vi "W08_T03_Judge.vi"() -> ()   [LabVIEW 2018]
doc: "Use this template to build a VI to use as a subVI."
panel:
  out "error out":errorcluster
  out "result":string
  out "value used":dbl
  in  "error in (no error)":errorcluster
  in  "true V (sim)":dbl
  in  "DMM loose (sim)":bool
  # "Read DMM.vi here is a fake (W08_sub). DMM loose (sim) and true V (sim) stand in for the real meter."
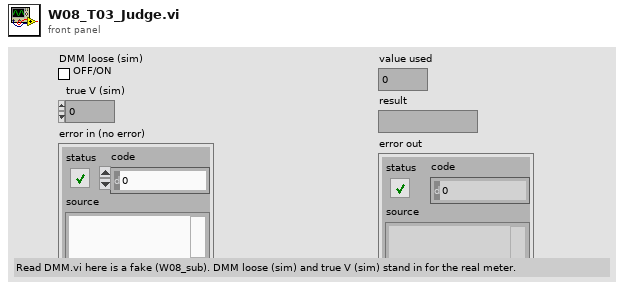
[diagram p1: front panel]
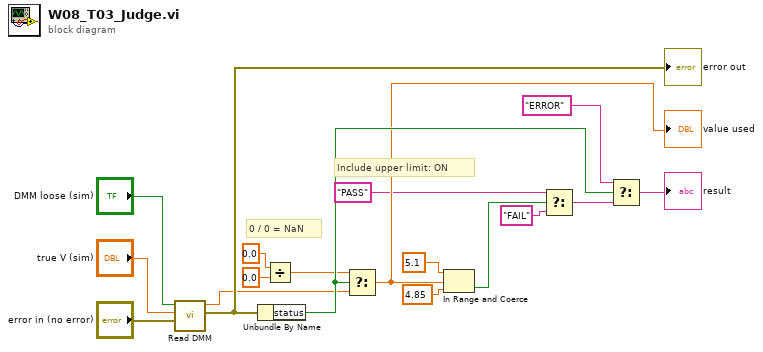
[diagram p0: block diagram]
diagram:
  # "Include upper limit: ON"
  # "0 / 0 = NaN"
  n1 = call "Read DMM.vi"("error in (no error)"="error in (no error)", "true V (sim)"="true V (sim)", "DMM loose (sim)"="DMM loose (sim)") -> ("error out"=w15:errorcluster, "reading"=w13:dbl)  [unwired: 7 in]
  "error out" <- w15
  n2 = Unbundle By Name(w15) -> ("status"=w14:bool)
  n3 = Divide(x=0.0, y=0.0) -> (x/y=w10:dbl)
  n4 = Select(t=w10, s=w14, f=w13) -> (s? t:f=w9:dbl)
  "value used" <- w9
  n5 = In Range and Coerce(upper limit=5.1, x=w9, lower limit=4.85) -> (In Range?=w6:bool)  [unwired: 1 out]
  n6 = Select(t="PASS", s=w6, f="FAIL") -> (s? t:f=w2:string)
  n7 = Select(t="ERROR", s=w14, f=w2) -> (s? t:f=→"result":string)
